vi "Trimming_Coil_Monitor.vi"() -> ()   [LabVIEW 2025]
panel:
  out "Cluster":T1
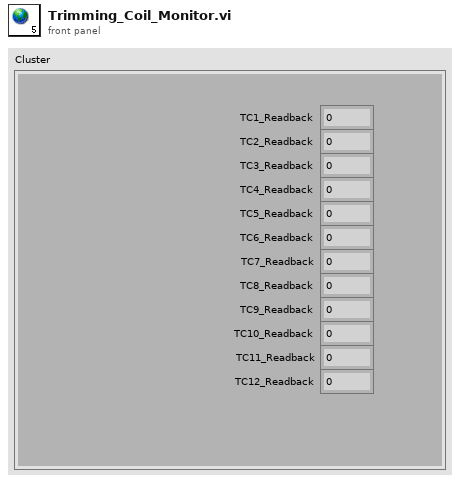
[diagram p1: front panel]
types:
  T1 = cluster{"TC1_Readback":dbl, "TC2_Readback":dbl, "TC3_Readback":dbl, "TC4_Readback":dbl, "TC5_Readback":dbl, "TC6_Readback":dbl, "TC7_Readback":dbl, "TC8_Readback":dbl, "TC9_Readback":dbl, "TC10_Readback":dbl, "TC11_Readback":dbl, "TC12_Readback":dbl}
diagram:
